vi "GetClassTemplates.vi"(0 "ClassWriterGOOP400 in":refnum<class "ClassWriterGOOP400.lvclass">, 1 "DerivedFromThisClass(if any)":refnum<vi>, 5 "error in (no error)":errorcluster) -> (14 "ClassWriterGOOP400 out":refnum<class "ClassWriterGOOP400.lvclass">, 15 "Templates(Matching Connector Pane Settings)":T1[](array[typedef]), 16 "AllTemplateNames(FolderNames)":string[](array[string]), 19 "error out":errorcluster)   [LabVIEW 2020, in "ClassWriterGOOP400.lvclass"]
uses:
  <resource>/Framework/Providers/Open_GDS/ClassProviders/Provider_EndevoGOOP400/ClassWriterGOOP400_class/ClassWriterGOOP400.lvclass
  <resource>/Framework/Providers/Open_GDS/ClassProviders/Provider_BaseClassInterface/ClassTemplateType.ctl
  <resource>/Framework/Providers/Open_GDS/ClassProviders/Provider_EndevoGOOP400/Templates/EndevoG4TemplateNames.ctl
  <resource>/Framework/Providers/Open_GDS/ClassProviders/Common/ScriptingFunctions/Scripting_ConnectorPanePatternType.ctl
  <resource>/Framework/Providers/Open_GDS/ClassProviders/Provider_EndevoGOOP400/ClassWriterGOOP400_class/ClassWriterGOOP400.lvclass/ClassWriterGOOP400.ctl
  <resource>/Framework/Providers/Open_GDS/ClassProviders/Provider_BaseClassInterface/ClassWriter_class/ClassWriter.lvclass
  <resource>/Framework/Providers/Open_GDS/ClassProviders/Provider_LvNativeClass/ClassWriterNative_class/ClassWriterNative.lvclass
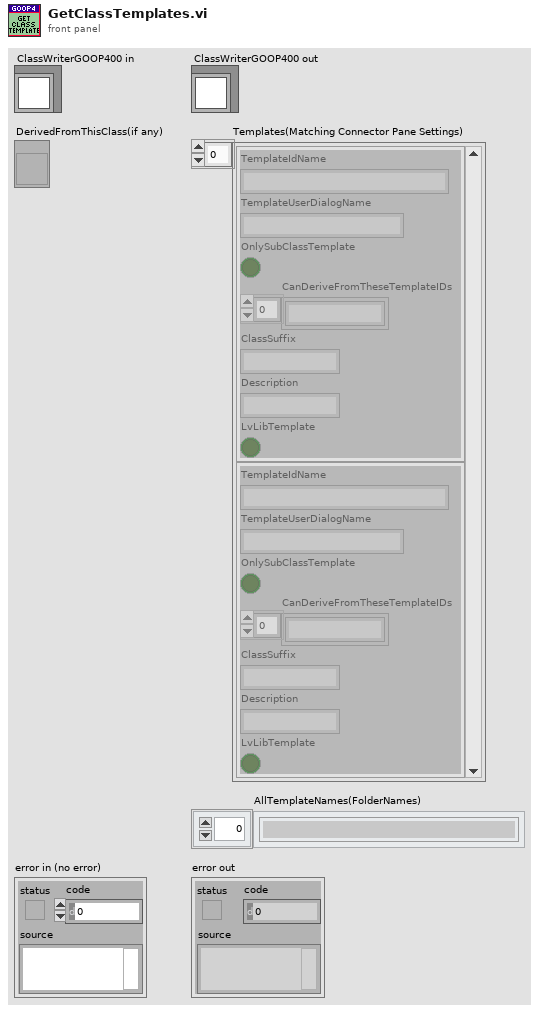
[diagram p1: front panel]
types:
  T1 = typedef "ClassWriter.lvclass/ClassTemplateType.ctl" = cluster{"TemplateIdName":string, "TemplateUserDialogName":string, "OnlySubClassTemplate":bool, "CanDeriveFromTheseTemplateIDs":string[], "ClassSuffix":string, "Description":string, "LvLibTemplate":bool}
  T2 = typedef "EndevoG4TemplateNames.ctl" = enum16{"G4BaseTemplate_Simple_4x4x4", "G4SubTemplate_Simple_4x4x4", "G4BaseTemplate_Simple_6x8x6", "G4SubTemplate_Simple_6x8x6", "G4BaseTemplate_Singleton_4x4x4", "G4SubTemplate_Singleton_4x4x4", "G4BaseTemplate_Singleton_6x8x6", "G4SubTemplate_Singleton_6x8x6", "G4InterfaceTemplate_6x8x6", "G4InterfaceTemplate_4x4x4", "G4BaseTemplate_Simple_5x6x5", "G4BaseTemplate_Singleton_5x6x5", "G4InterfaceTemplate_5x6x5", "G4SubTemplate_Simple_5x6x5", "G4SubTemplate_Singleton_5x6x5"}
  T3 = typedef "Scripting_ConnectorPanePatternType.ctl" = u16
  T4 = typedef "GDSLvCLass_ClassSettingsType.ctl" = cluster{"ClassProviderName":string, "ClassTemplateUsed":string, "ClassTemplateVersion":string, "ClassDescription":string, "PlugIns":T5[], "ConnectorPanePattern":string}
  T5 = typedef "GDSLvClass_PlugIn.ctl" = cluster{"Type":T6, "ID":string, "Version":string, "Path":path, "Name":string, "Data":variant}
  T6 = typedef "GDSLvClass_PlugInTypes.ctl" = enum16{"DesignPattern", "MethodTypes"}
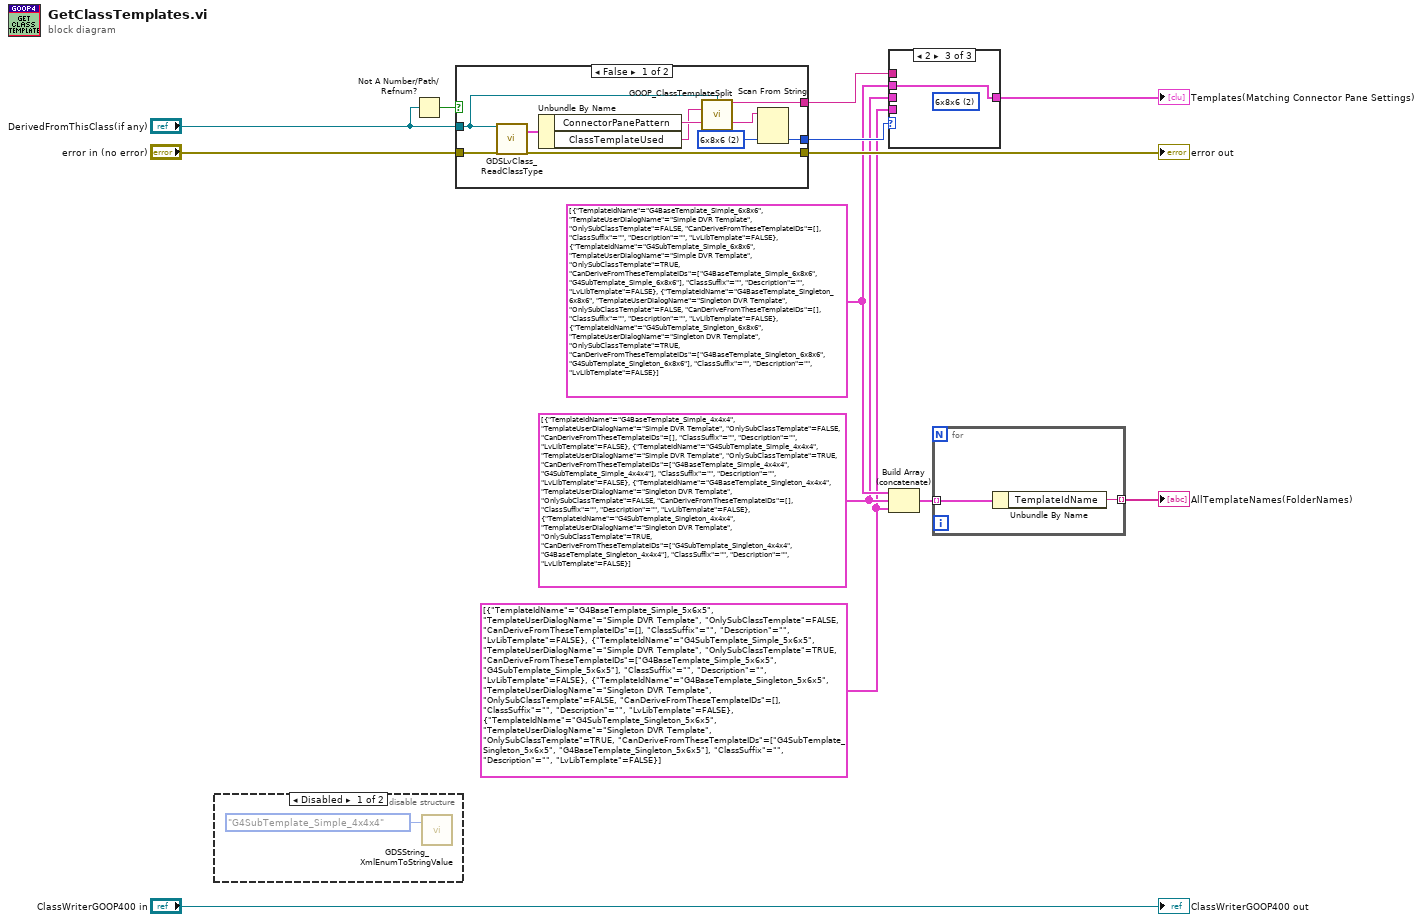
[diagram p0: block diagram]
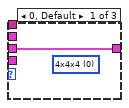
[diagram p3: hidden frame]
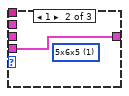
[diagram p4: hidden frame]
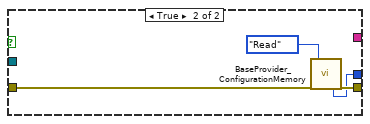
[diagram p5: hidden frame]
diagram:
  w4 = T1[] [{"TemplateIdName"="G4BaseTemplate_Simple_6x8x6", "TemplateUserDialogName"="Simple DVR Template", "OnlySubClassTemplate"=FALSE, "CanDeriveFromTheseTemplateIDs"=[], "ClassSuffix"="", "Description"="", "LvLibTemplate"=FALSE}, {"TemplateIdName"="G4SubTemplate_Simple_6x8x6", "TemplateUserDialogName"="Simple DVR Template", "OnlySubClassTemplate"=TRUE, "CanDeriveFromTheseTemplateIDs"=["G4BaseTemplate_Simple_6x8x6", "G4SubTemplate_Simple_6x8x6"], "ClassSuffix"="", "Description"="", "LvLibTemplate"=FALSE}, {"TemplateIdName"="G4BaseTemplate_Singleton_6x8x6", "TemplateUserDialogName"="Singleton DVR Template", "OnlySubClassTemplate"=FALSE, "CanDeriveFromTheseTemplateIDs"=[], "ClassSuffix"="", "Description"="", "LvLibTemplate"=FALSE}, {"TemplateIdName"="G4SubTemplate_Singleton_6x8x6", "TemplateUserDialogName"="Singleton DVR Template", "OnlySubClassTemplate"=TRUE, "CanDeriveFromTheseTemplateIDs"=["G4BaseTemplate_Singleton_6x8x6", "G4SubTemplate_Singleton_6x8x6"], "ClassSuffix"="", "Description"="", "LvLibTemplate"=FALSE}] ("TemplateIdNames")
  w2 = T1[] [{"TemplateIdName"="G4BaseTemplate_Simple_5x6x5", "TemplateUserDialogName"="Simple DVR Template", "OnlySubClassTemplate"=FALSE, "CanDeriveFromTheseTemplateIDs"=[], "ClassSuffix"="", "Description"="", "LvLibTemplate"=FALSE}, {"TemplateIdName"="G4SubTemplate_Simple_5x6x5", "TemplateUserDialogName"="Simple DVR Template", "OnlySubClassTemplate"=TRUE, "CanDeriveFromTheseTemplateIDs"=["G4BaseTemplate_Simple_5x6x5", "G4SubTemplate_Simple_5x6x5"], "ClassSuffix"="", "Description"="", "LvLibTemplate"=FALSE}, {"TemplateIdName"="G4BaseTemplate_Singleton_5x6x5", "TemplateUserDialogName"="Singleton DVR Template", "OnlySubClassTemplate"=FALSE, "CanDeriveFromTheseTemplateIDs"=[], "ClassSuffix"="", "Description"="", "LvLibTemplate"=FALSE}, {"TemplateIdName"="G4SubTemplate_Singleton_5x6x5", "TemplateUserDialogName"="Singleton DVR Template", "OnlySubClassTemplate"=TRUE, "CanDeriveFromTheseTemplateIDs"=["G4SubTemplate_Singleton_5x6x5", "G4BaseTemplate_Singleton_5x6x5"], "ClassSuffix"="", "Description"="", "LvLibTemplate"=FALSE}] ("TemplateIdNames")
  w3 = T1[] [{"TemplateIdName"="G4BaseTemplate_Simple_4x4x4", "TemplateUserDialogName"="Simple DVR Template", "OnlySubClassTemplate"=FALSE, "CanDeriveFromTheseTemplateIDs"=[], "ClassSuffix"="", "Description"="", "LvLibTemplate"=FALSE}, {"TemplateIdName"="G4SubTemplate_Simple_4x4x4", "TemplateUserDialogName"="Simple DVR Template", "OnlySubClassTemplate"=TRUE, "CanDeriveFromTheseTemplateIDs"=["G4BaseTemplate_Simple_4x4x4", "G4SubTemplate_Simple_4x4x4"], "ClassSuffix"="", "Description"="", "LvLibTemplate"=FALSE}, {"TemplateIdName"="G4BaseTemplate_Singleton_4x4x4", "TemplateUserDialogName"="Singleton DVR Template", "OnlySubClassTemplate"=FALSE, "CanDeriveFromTheseTemplateIDs"=[], "ClassSuffix"="", "Description"="", "LvLibTemplate"=FALSE}, {"TemplateIdName"="G4SubTemplate_Singleton_4x4x4", "TemplateUserDialogName"="Singleton DVR Template", "OnlySubClassTemplate"=TRUE, "CanDeriveFromTheseTemplateIDs"=["G4SubTemplate_Singleton_4x4x4", "G4BaseTemplate_Singleton_4x4x4"], "ClassSuffix"="", "Description"="", "LvLibTemplate"=FALSE}] ("TemplateIdNames")
  n1 = disable-structure shown="Disabled" {
    frame Disabled {
      n2 = call <resource>:"GDSString_XmlEnumToStringValue.vi"("EnumVariantIn(used if String is Empty)"=EndevoG4TemplateNames."G4SubTemplate_Simple_4x4x4" ("TemplateNames")) -> ()  [unwired: 15 in, 4 out]
    }
    frame Enabled {
    }
  }
  n3 = Not A Number/Path/Refnum?(number/path/refnum="DerivedFromThisClass(if any)") -> (NaN/Path/Refnum?=w12:bool)
  n4 = case shown="False" w12 {
    tunnel: "error in (no error)" -> [w20 w26]
    tunnel: "DerivedFromThisClass(if any)" -> [w15 _]
    tunnel: [w19 w25] -> w8
    tunnel: [w18 w24] -> w11
    tunnel: [w16 _] -> w7
    frame False {
      w21 = T3 2 items=["4x4x4", "5x6x5", "6x8x6"] ("Pattern")
      n5 = call <resource>:"GDSLvClass_ReadClassType.vi"("Class Refnum In"=w15, "error in (no error)"=w20) -> ("ClassSettings"=w23:T4, "error out"=w19:errorcluster)  [unwired: 15 in, 1 out]
      n6 = Unbundle By Name(w23) -> ("ConnectorPanePattern"=w22:string, "ClassTemplateUsed"=w17:string)
      n7 = call <resource>:"GOOP_ClassTemplateSplit.vi"("ClassItemRefIn"=w15, "FullClassTemplate"=w17) -> ("StandardTemplate"=w16:string)  [unwired: 12 in, 1 out]
      n8 = Scan From String(input string=w22, default 1=w21) -> (output 1=w18:T3)  [unwired: 3 in, 3 out]
    }
    frame True {
      n9 = call <resource>:"BaseProvider_ConfigurationMemory.vi"("error in (no error)"=w26, "Action"=enum16{"Read", "Load", "Save"}."Read") -> ("PatternOut"=w24:T3, "error out"=w25:errorcluster)  [unwired: 11 in, 5 out]
    }
  }
  "error out" <- w8
  n10 = case shown="2" w11 {
    tunnel: [w28 w29 w30] -> w6
    tunnel: w7 -> [_ _ _]
    tunnel: w3 -> [w28 _ _]
    tunnel: w2 -> [_ w29 _]
    tunnel: w4 -> [_ _ w30]
    frame 0, Default {
      (unwired) T3 0 items=["4x4x4", "5x6x5", "6x8x6"] ("Pattern")
    }
    frame 1 {
      (unwired) T3 1 items=["4x4x4", "5x6x5", "6x8x6"] ("Pattern")
    }
    frame 2 {
      (unwired) T3 2 items=["4x4x4", "5x6x5", "6x8x6"] ("Pattern")
    }
  }
  "Templates(Matching Connector Pane Settings)" <- w6
  n11 = Build Array (concatenate)(w4, w3, w2) -> (w5:T1[])
  n12 = for {
    tunnel: w5 -> [w32] mode=indexing
    tunnel: [w31] -> w1 mode=indexing
    n13 = Unbundle By Name(w32) -> ("TemplateIdName"=w31:string)
  }
  "AllTemplateNames(FolderNames)" <- w1
  "ClassWriterGOOP400 out" <- "ClassWriterGOOP400 in"
